vi "PicoScopeospaExampleRapidBlockBulkOverlapped_jittertimes.vi"() -> ()   [LabVIEW 2010]
uses:
  shared/PicoBuffers.ctl
  <vilib>/Waveform/DWDTOps.llb/DWDT Analog to Digital.vi
  PicoScopepsospaLib/PicoScopeospaDigitalChannelSettings.ctl
  PicoScopepsospaLib/PicoScopeospaAnalogChannelSettings.ctl
  shared/Buffer and Transfer Settings.ctl
  shared/Acquisition Settings.ctl
  shared/Segment Range.ctl
panel:
  out "nCaptures live":u64
  out "nCaptures":u64
  out "Trigger Info":T1(array[cluster])
  in  "timeIntervalRequested":dbl=2e-10 format="%#6_6p"
  in  "Write to file":bool
  in  "Channels":T2={"Channel A Settings "={"Enabled"=TRUE, "Coupling"=1, "Range"=8, "Analogue Offset"=0.0, "BandWidth"=0, "PROBE_RANGE_INFO"=0}, "Channel B Settings "={"Enabled"=FALSE, "Coupling"=1, "Range"=8, "Analogue Offset"=0.0, "BandWidth"=0, "PROBE_RANGE_INFO"=0}, "Channel C Settings "={"Enabled"=FALSE, "Coupling"=1, "Range"=8, "Analogue Offset"=0.0, "BandWidth"=0, "PROBE_RANGE_INFO"=0}, "Channel D Settings "={"Enabled"=FALSE, "Coupling"=1, "Range"=8, "Analogue Offset"=0.0, "BandWidth"=0, "PROBE_RANGE_INFO"=0}, "Channel E Settings "={"Enabled"=FALSE, "Coupling"=50, "Range"=5, "Analogue Offset"=0.0, "BandWidth"=0, "PROBE_RANGE_INFO"=0}, "Channel F Settings "={"Enabled"=FALSE, "Coupling"=50, "Range"=5, "Analogue Offset"=0.0, "BandWidth"=0, "PROBE_RANGE_INFO"=0}, "Channel G Settings "={"Enabled"=FALSE, "Coupling"=50, "Range"=5, "Analogue Offset"=0.0, "BandWidth"=0, "PROBE_RANGE_INFO"=0}, "Channel H Settings "={"Enabled"=FALSE, "Coupling"=50, "Range"=5, "Analogue Offset"=0.0, "BandWidth"=0, "PROBE_RANGE_INFO"=0}} {"Channel H Settings"."PROBE_RANGE_INFO" items=["PROBE_NONE_NV"=0, "X1_PROBE_NV"=1, "X10_PROBE_NV"=10]; "Channel H Settings"."BandWidth" items=["Full"=0, "100kHz"=100000, "20kHz"=200000, "1MHz"=1000000, "20MHz"=20000000, "25MHz"=25000000, "50MHz"=50000000, "200MHz"=200000000, "250MHz"=250000000, "500MHz"=500000000]; "Channel H Settings"."Range" items=["10mV"=0, "20mV"=1, "50mV"=2, "100mV"=3, "200mV"=4, "500mV"=5, "1V"=6, "2V"=7, "5V"=8, "10V"=9, "20V"=10, "50V"=11, "100V"=12, "200V"=13, "x10_Probe_100mV"=32, "x10_Probe_200mV"=33, "x10_Probe_500mV"=34, "x10_Probe_1V"=35, "x10_Probe_2V"=36, "x10_Probe_5V"=37, "x10_Probe_10V"=38, "x10_Probe_20V"=39, "x10_Probe_50V"=40, "x10_Probe_100V"=41, "x10_Probe_200V"=42, "x10_Probe_500V"=43, "CURRENT_CLAMP_60A_2A"=10500, "CURRENT_CLAMP_60A_5A"=10501, "CURRENT_CLAMP_60A_10A"=10502, "CURRENT_CLAMP_60A_20A"=10503, "CURRENT_CLAMP_60A_50A"=10504, "CURRENT_CLAMP_60A_60A"=10505, "CURRENT_CLAMP_60A_V2_0_5A"=10600, "CURRENT_CLAMP_60A_V2_1A"=10601, "CURRENT_CLAMP_60A_V2_2A"=10602, "CURRENT_CLAMP_60A_V2_5A"=10603, "CURRENT_CLAMP_60A_V2_10A"=10604, "CURRENT_CLAMP_60A_V2_20A"=10605, "CURRENT_CLAMP_60A_V2_50A"=10606, "CURRENT_CLAMP_60A_V2_60A"=10607, "RESISTANCE_LEAD_NEG5_TO_20OHM"=7000, "RESISTANCE_LEAD_NEG50_TO_200OHM"=7001, "RESISTANCE_LEAD_NEG500_TO_2KOHM"=7002, "RESISTANCE_LEAD_NEG5K_TO_20KOHM"=7003, "RESISTANCE_LEAD_NEG50K_TO_LEAD_200KOHM"=7004, "RESISTANCE_LEAD_NEG500K_TO_LEAD_2MOHM"=7005, "RESISTANCE_LEAD_DIODE_TEST"=7006, "HT_NEG3_TO_5KV"=8950, "HT_NEG3_TO_10KV"=8951, "HT_NEG5_TO_20KV"=8952, "HT_NEG5_TO_50KV"=8953, "HT_NEG5_TO_100KV"=8954, "HT_NEG3_TO_5KV_INVERTED"=8955, "HT_NEG3_TO_10KV_INVERTED"=8956, "HT_NEG5_TO_20KV_INVERTED"=8957, "HT_NEG5_TO_50KV_INVERTED"=8958, "HT_NEG5_TO_100KV_INVERTED"=8959, "TEMPERATURE_NEG50_TO_150DEGC"=9000, "PRESSURE_SENSOR_-100k-150k_PASCALS"=9100, "PRESSURE_SENSOR_-100k_TO_400k_PASCALS"=9101, "PRESSURE_SENSOR_-200k_TO_800k_PASCALS"=9102, "PRESSURE_SENSOR_-400k_TO_1600k_PASCALS"=9103, "PRESSURE_SENSOR_-400k_TO_3400k_PASCALS"=9104, "PRESSURE_SENSOR_-150k_TO_1350k_PASCALS"=9105]; "Channel H Settings"."Coupling" items=["AC"=0, "DC 1M Ohm"=1, "DC 50 Ohm"=50]; "Channel G Settings"."PROBE_RANGE_INFO" items=["PROBE_NONE_NV"=0, "X1_PROBE_NV"=1, "X10_PROBE_NV"=10]; "Channel G Settings"."BandWidth" items=["Full"=0, "100kHz"=100000, "20kHz"=200000, "1MHz"=1000000, "20MHz"=20000000, "25MHz"=25000000, "50MHz"=50000000, "200MHz"=200000000, "250MHz"=250000000, "500MHz"=500000000]; "Channel G Settings"."Range" items=["10mV"=0, "20mV"=1, "50mV"=2, "100mV"=3, "200mV"=4, "500mV"=5, "1V"=6, "2V"=7, "5V"=8, "10V"=9, "20V"=10, "50V"=11, "100V"=12, "200V"=13, "x10_Probe_100mV"=32, "x10_Probe_200mV"=33, "x10_Probe_500mV"=34, "x10_Probe_1V"=35, "x10_Probe_2V"=36, "x10_Probe_5V"=37, "x10_Probe_10V"=38, "x10_Probe_20V"=39, "x10_Probe_50V"=40, "x10_Probe_100V"=41, "x10_Probe_200V"=42, "x10_Probe_500V"=43, "CURRENT_CLAMP_60A_2A"=10500, "CURRENT_CLAMP_60A_5A"=10501, "CURRENT_CLAMP_60A_10A"=10502, "CURRENT_CLAMP_60A_20A"=10503, "CURRENT_CLAMP_60A_50A"=10504, "CURRENT_CLAMP_60A_60A"=10505, "CURRENT_CLAMP_60A_V2_0_5A"=10600, "CURRENT_CLAMP_60A_V2_1A"=10601, "CURRENT_CLAMP_60A_V2_2A"=10602, "CURRENT_CLAMP_60A_V2_5A"=10603, "CURRENT_CLAMP_60A_V2_10A"=10604, "CURRENT_CLAMP_60A_V2_20A"=10605, "CURRENT_CLAMP_60A_V2_50A"=10606, "CURRENT_CLAMP_60A_V2_60A"=10607, "RESISTANCE_LEAD_NEG5_TO_20OHM"=7000, "RESISTANCE_LEAD_NEG50_TO_200OHM"=7001, "RESISTANCE_LEAD_NEG500_TO_2KOHM"=7002, "RESISTANCE_LEAD_NEG5K_TO_20KOHM"=7003, "RESISTANCE_LEAD_NEG50K_TO_LEAD_200KOHM"=7004, "RESISTANCE_LEAD_NEG500K_TO_LEAD_2MOHM"=7005, "RESISTANCE_LEAD_DIODE_TEST"=7006, "HT_NEG3_TO_5KV"=8950, "HT_NEG3_TO_10KV"=8951, "HT_NEG5_TO_20KV"=8952, "HT_NEG5_TO_50KV"=8953, "HT_NEG5_TO_100KV"=8954, "HT_NEG3_TO_5KV_INVERTED"=8955, "HT_NEG3_TO_10KV_INVERTED"=8956, "HT_NEG5_TO_20KV_INVERTED"=8957, "HT_NEG5_TO_50KV_INVERTED"=8958, "HT_NEG5_TO_100KV_INVERTED"=8959, "TEMPERATURE_NEG50_TO_150DEGC"=9000, "PRESSURE_SENSOR_-100k-150k_PASCALS"=9100, "PRESSURE_SENSOR_-100k_TO_400k_PASCALS"=9101, "PRESSURE_SENSOR_-200k_TO_800k_PASCALS"=9102, "PRESSURE_SENSOR_-400k_TO_1600k_PASCALS"=9103, "PRESSURE_SENSOR_-400k_TO_3400k_PASCALS"=9104, "PRESSURE_SENSOR_-150k_TO_1350k_PASCALS"=9105]; "Channel G Settings"."Coupling" items=["AC"=0, "DC 1M Ohm"=1, "DC 50 Ohm"=50]; "Channel F Settings"."PROBE_RANGE_INFO" items=["PROBE_NONE_NV"=0, "X1_PROBE_NV"=1, "X10_PROBE_NV"=10]; "Channel F Settings"."BandWidth" items=["Full"=0, "100kHz"=100000, "20kHz"=200000, "1MHz"=1000000, "20MHz"=20000000, "25MHz"=25000000, "50MHz"=50000000, "200MHz"=200000000, "250MHz"=250000000, "500MHz"=500000000]; "Channel F Settings"."Range" items=["10mV"=0, "20mV"=1, "50mV"=2, "100mV"=3, "200mV"=4, "500mV"=5, "1V"=6, "2V"=7, "5V"=8, "10V"=9, "20V"=10, "50V"=11, "100V"=12, "200V"=13, "x10_Probe_100mV"=32, "x10_Probe_200mV"=33, "x10_Probe_500mV"=34, "x10_Probe_1V"=35, "x10_Probe_2V"=36, "x10_Probe_5V"=37, "x10_Probe_10V"=38, "x10_Probe_20V"=39, "x10_Probe_50V"=40, "x10_Probe_100V"=41, "x10_Probe_200V"=42, "x10_Probe_500V"=43, "CURRENT_CLAMP_60A_2A"=10500, "CURRENT_CLAMP_60A_5A"=10501, "CURRENT_CLAMP_60A_10A"=10502, "CURRENT_CLAMP_60A_20A"=10503, "CURRENT_CLAMP_60A_50A"=10504, "CURRENT_CLAMP_60A_60A"=10505, "CURRENT_CLAMP_60A_V2_0_5A"=10600, "CURRENT_CLAMP_60A_V2_1A"=10601, "CURRENT_CLAMP_60A_V2_2A"=10602, "CURRENT_CLAMP_60A_V2_5A"=10603, "CURRENT_CLAMP_60A_V2_10A"=10604, "CURRENT_CLAMP_60A_V2_20A"=10605, "CURRENT_CLAMP_60A_V2_50A"=10606, "CURRENT_CLAMP_60A_V2_60A"=10607, "RESISTANCE_LEAD_NEG5_TO_20OHM"=7000, "RESISTANCE_LEAD_NEG50_TO_200OHM"=7001, "RESISTANCE_LEAD_NEG500_TO_2KOHM"=7002, "RESISTANCE_LEAD_NEG5K_TO_20KOHM"=7003, "RESISTANCE_LEAD_NEG50K_TO_LEAD_200KOHM"=7004, "RESISTANCE_LEAD_NEG500K_TO_LEAD_2MOHM"=7005, "RESISTANCE_LEAD_DIODE_TEST"=7006, "HT_NEG3_TO_5KV"=8950, "HT_NEG3_TO_10KV"=8951, "HT_NEG5_TO_20KV"=8952, "HT_NEG5_TO_50KV"=8953, "HT_NEG5_TO_100KV"=8954, "HT_NEG3_TO_5KV_INVERTED"=8955, "HT_NEG3_TO_10KV_INVERTED"=8956, "HT_NEG5_TO_20KV_INVERTED"=8957, "HT_NEG5_TO_50KV_INVERTED"=8958, "HT_NEG5_TO_100KV_INVERTED"=8959, "TEMPERATURE_NEG50_TO_150DEGC"=9000, "PRESSURE_SENSOR_-100k-150k_PASCALS"=9100, "PRESSURE_SENSOR_-100k_TO_400k_PASCALS"=9101, "PRESSURE_SENSOR_-200k_TO_800k_PASCALS"=9102, "PRESSURE_SENSOR_-400k_TO_1600k_PASCALS"=9103, "PRESSURE_SENSOR_-400k_TO_3400k_PASCALS"=9104, "PRESSURE_SENSOR_-150k_TO_1350k_PASCALS"=9105]; "Channel F Settings"."Coupling" items=["AC"=0, "DC 1M Ohm"=1, "DC 50 Ohm"=50]; "Channel E Settings"."PROBE_RANGE_INFO" items=["PROBE_NONE_NV"=0, "X1_PROBE_NV"=1, "X10_PROBE_NV"=10]; "Channel E Settings"."BandWidth" items=["Full"=0, "100kHz"=100000, "20kHz"=200000, "1MHz"=1000000, "20MHz"=20000000, "25MHz"=25000000, "50MHz"=50000000, "200MHz"=200000000, "250MHz"=250000000, "500MHz"=500000000]; "Channel E Settings"."Range" items=["10mV"=0, "20mV"=1, "50mV"=2, "100mV"=3, "200mV"=4, "500mV"=5, "1V"=6, "2V"=7, "5V"=8, "10V"=9, "20V"=10, "50V"=11, "100V"=12, "200V"=13, "x10_Probe_100mV"=32, "x10_Probe_200mV"=33, "x10_Probe_500mV"=34, "x10_Probe_1V"=35, "x10_Probe_2V"=36, "x10_Probe_5V"=37, "x10_Probe_10V"=38, "x10_Probe_20V"=39, "x10_Probe_50V"=40, "x10_Probe_100V"=41, "x10_Probe_200V"=42, "x10_Probe_500V"=43, "CURRENT_CLAMP_60A_2A"=10500, "CURRENT_CLAMP_60A_5A"=10501, "CURRENT_CLAMP_60A_10A"=10502, "CURRENT_CLAMP_60A_20A"=10503, "CURRENT_CLAMP_60A_50A"=10504, "CURRENT_CLAMP_60A_60A"=10505, "CURRENT_CLAMP_60A_V2_0_5A"=10600, "CURRENT_CLAMP_60A_V2_1A"=10601, "CURRENT_CLAMP_60A_V2_2A"=10602, "CURRENT_CLAMP_60A_V2_5A"=10603, "CURRENT_CLAMP_60A_V2_10A"=10604, "CURRENT_CLAMP_60A_V2_20A"=10605, "CURRENT_CLAMP_60A_V2_50A"=10606, "CURRENT_CLAMP_60A_V2_60A"=10607, "RESISTANCE_LEAD_NEG5_TO_20OHM"=7000, "RESISTANCE_LEAD_NEG50_TO_200OHM"=7001, "RESISTANCE_LEAD_NEG500_TO_2KOHM"=7002, "RESISTANCE_LEAD_NEG5K_TO_20KOHM"=7003, "RESISTANCE_LEAD_NEG50K_TO_LEAD_200KOHM"=7004, "RESISTANCE_LEAD_NEG500K_TO_LEAD_2MOHM"=7005, "RESISTANCE_LEAD_DIODE_TEST"=7006, "HT_NEG3_TO_5KV"=8950, "HT_NEG3_TO_10KV"=8951, "HT_NEG5_TO_20KV"=8952, "HT_NEG5_TO_50KV"=8953, "HT_NEG5_TO_100KV"=8954, "HT_NEG3_TO_5KV_INVERTED"=8955, "HT_NEG3_TO_10KV_INVERTED"=8956, "HT_NEG5_TO_20KV_INVERTED"=8957, "HT_NEG5_TO_50KV_INVERTED"=8958, "HT_NEG5_TO_100KV_INVERTED"=8959, "TEMPERATURE_NEG50_TO_150DEGC"=9000, "PRESSURE_SENSOR_-100k-150k_PASCALS"=9100, "PRESSURE_SENSOR_-100k_TO_400k_PASCALS"=9101, "PRESSURE_SENSOR_-200k_TO_800k_PASCALS"=9102, "PRESSURE_SENSOR_-400k_TO_1600k_PASCALS"=9103, "PRESSURE_SENSOR_-400k_TO_3400k_PASCALS"=9104, "PRESSURE_SENSOR_-150k_TO_1350k_PASCALS"=9105]; "Channel E Settings"."Coupling" items=["AC"=0, "DC 1M Ohm"=1, "DC 50 Ohm"=50]; "Channel D Settings"."BandWidth" items=["Full"=0, "100kHz"=100000, "20kHz"=200000, "1MHz"=1000000, "20MHz"=20000000, "25MHz"=25000000, "50MHz"=50000000, "100MHz"=100000000, "200MHz"=200000000, "250MHz"=250000000, "350MHz"=350000000, "500MHz"=500000000]; "Channel D Settings"."PROBE_RANGE_INFO" items=["PROBE_NONE_NV"=0, "X1_PROBE_NV"=1, "X10_PROBE_NV"=10]; "Channel D Settings"."Range" items=["10mV", "20mV", "50mV", "100mV", "200mV", "500mV", "1V", "2V", "5V", "10V", "20V", "50V", "100V", "200V"]; "Channel D Settings"."Coupling" items=["AC"=0, "DC 1M Ohm"=1, "DC 50 Ohm"=50]; "Channel C Settings"."BandWidth" items=["Full"=0, "100kHz"=100000, "20kHz"=200000, "1MHz"=1000000, "20MHz"=20000000, "25MHz"=25000000, "50MHz"=50000000, "100MHz"=100000000, "200MHz"=200000000, "250MHz"=250000000, "350MHz"=350000000, "500MHz"=500000000]; "Channel C Settings"."PROBE_RANGE_INFO" items=["PROBE_NONE_NV"=0, "X1_PROBE_NV"=1, "X10_PROBE_NV"=10]; "Channel C Settings"."Range" items=["10mV", "20mV", "50mV", "100mV", "200mV", "500mV", "1V", "2V", "5V", "10V", "20V", "50V", "100V", "200V"]; "Channel C Settings"."Coupling" items=["AC"=0, "DC 1M Ohm"=1, "DC 50 Ohm"=50]; "Channel B Settings"."BandWidth" items=["Full"=0, "100kHz"=100000, "20kHz"=200000, "1MHz"=1000000, "20MHz"=20000000, "25MHz"=25000000, "50MHz"=50000000, "100MHz"=100000000, "200MHz"=200000000, "250MHz"=250000000, "350MHz"=350000000, "500MHz"=500000000]; "Channel B Settings"."PROBE_RANGE_INFO" items=["PROBE_NONE_NV"=0, "X1_PROBE_NV"=1, "X10_PROBE_NV"=10]; "Channel B Settings"."Range" items=["10mV", "20mV", "50mV", "100mV", "200mV", "500mV", "1V", "2V", "5V", "10V", "20V", "50V", "100V", "200V"]; "Channel B Settings"."Coupling" items=["AC"=0, "DC 1M Ohm"=1, "DC 50 Ohm"=50]; "Channel A Settings"."PROBE_RANGE_INFO" items=["PROBE_NONE_NV"=0, "X1_PROBE_NV"=1, "X10_PROBE_NV"=10]; "Channel A Settings"."Range" items=["10mV", "20mV", "50mV", "100mV", "200mV", "500mV", "1V", "2V", "5V", "10V", "20V", "50V", "100V", "200V"]; "Channel A Settings"."BandWidth" items=["Full"=0, "100kHz"=100000, "20kHz"=200000, "1MHz"=1000000, "20MHz"=20000000, "25MHz"=25000000, "50MHz"=50000000, "100MHz"=100000000, "200MHz"=200000000, "250MHz"=250000000, "350MHz"=350000000, "500MHz"=500000000]; "Channel A Settings"."Coupling" items=["AC"=0, "DC 1M Ohm"=1, "DC 50 Ohm"=50]}
  out "overflow":i16[](array[numeric])=[1023] format="%010d"
  out "Trigger Offsets":cluster{"Samples":u64, "Time (seconds)":dbl}[](array[cluster]) {"Time (seconds)" format="%#_5p"}
  in  "Stop Display":bool
  out "Capture Complete":bool
  in  "Run":bool
  in  "Display Buffer Index":i32
  in  "Segment Range":T3={"fromSegmentIndex"=0, "toSegmentIndex"=9} {"toSegmentIndex" format="%.4p"; "fromSegmentIndex" format="%.4p"}
  in  "nSegments":u64=10 format="%.4p"
  out "error out":errorcluster
  in  "Data file":path=path "PicoScopeospaExampleRapidBlock ChA Data"
  in  "Digital Channels":T4={"Port 0 Settings "={"Enabled"=FALSE, "Threshold Level (Volts)"=3.0}, "Port 1 Settings"={"Enabled"=FALSE, "Threshold Level (Volts)"=3.0}} {"Port 1 Settings"."Threshold Level (Volts)" format="%#_4p"; "Port 0 Settings"."Threshold Level (Volts)" format="%#_4p"}
  in  "Trigger Settings":T5={"Trigger Enabled"=FALSE, "Trigger Threshold (Volts)"=0.0, "Trigger Direction"=2, "Trigger Delay (samples)"=0, "Auto Trigger Time (us)"=1000000, "Trigger Source"=0} {"Trigger Source" items=["Channel A"=0, "Channel B"=1, "Channel C"=2, "Channel D"=3, "Channel E"=4, "Channel F"=5, "Channel G"=6, "Channel H"=7, "Port 0"=128, "Port 1"=129, "Trigger AUX"=1001]; "Auto Trigger Time (us)" format="%.4p"; "Trigger Direction" items=["Above", "Below", "Rising", "Falling", "Rising or Falling"]; "Trigger Threshold (Volts)" format="%#_6p"}
  in  "Buffer and Transfer Settings":T6={"startIndex"=0, "Samples"=10000000, "Down Sample Ratio"=10, "Down-Sample Mode"=2147483648} {"Down-Sample Mode" items=["RAW none"=2147483648, "None"=0, "Aggregate"=1, "Decimate"=2, "Average"=4]; "Down Sample Ratio" step=1; "Samples" format="%_6p"}
  in  "Acquisition Settings":T7={"preTriggerSamples"=0, "postTriggerSamples"=10000000, "timebase"=5} {"postTriggerSamples" format="%_6p"; "preTriggerSamples" format="%_6p"}
  out "Properties Panel":T8 {"Max Total Capture Time Available (sec)" format="%.3p"; "Sample Frequency" format="%.6p"; "Sample Rate" format="%.3p"; "Max Samples Available" format="%_6p"; "Total Capture Time (sec)" format="%.3p"}
  out "Port 0":digitalwaveform(graph)={"t0"=timestamp(0 s since 1904-01-01), "dt"=8e-09, "Y"={"transitions"=[], "data"=[]}}
  in  "stop":bool
  out "Analog Channels":cluster{i32, dbl, "Data":dbl[]}[](graph)
  out "Device Info":T9={"PICO_DRIVER_VERSION"="", "PICO_USB_VERSION"="", "PICO_HARDWARE_VERSION"="", "PICO_VARIANT_INFO"="", "PICO_BATCH_AND_SERIAL"="", "PICO_CAL_DATE"="", "PICO_KERNEL_VERSION"="", "PICO_DIGITAL_HARDWARE_VERSION"="", "PICO_ANALOGUE_HARDWARE_VERSION"="", "PICO_FIRMWARE_VERSION_1"="", "PICO_FIRMWARE_VERSION_2"="", "PICO_IPP_VERSION"="", "PICO_DRIVER_PATH"="", "PICO_FIRMWARE_VERSION_3"="", "PICO_FRONT_PANEL_FIRMWARE_VERSION"="", "Number of Channels"=8, "MSO"=FALSE}
  out "Pico ospa Units":string
  in  "Resolution":u32(ring)=10 items=["8-bit"=0, "12-bit"=1, "14-bit"=2, "15-bit"=3, "16-bit"=4, "10-bit"=10]
  in  "Serial Number":string
  in  "Use Serial Number":bool
  in  "error in (no error)":errorcluster
  # "Bit 0 = ChA"
  # "D8-D15"
  # "DO-D7"
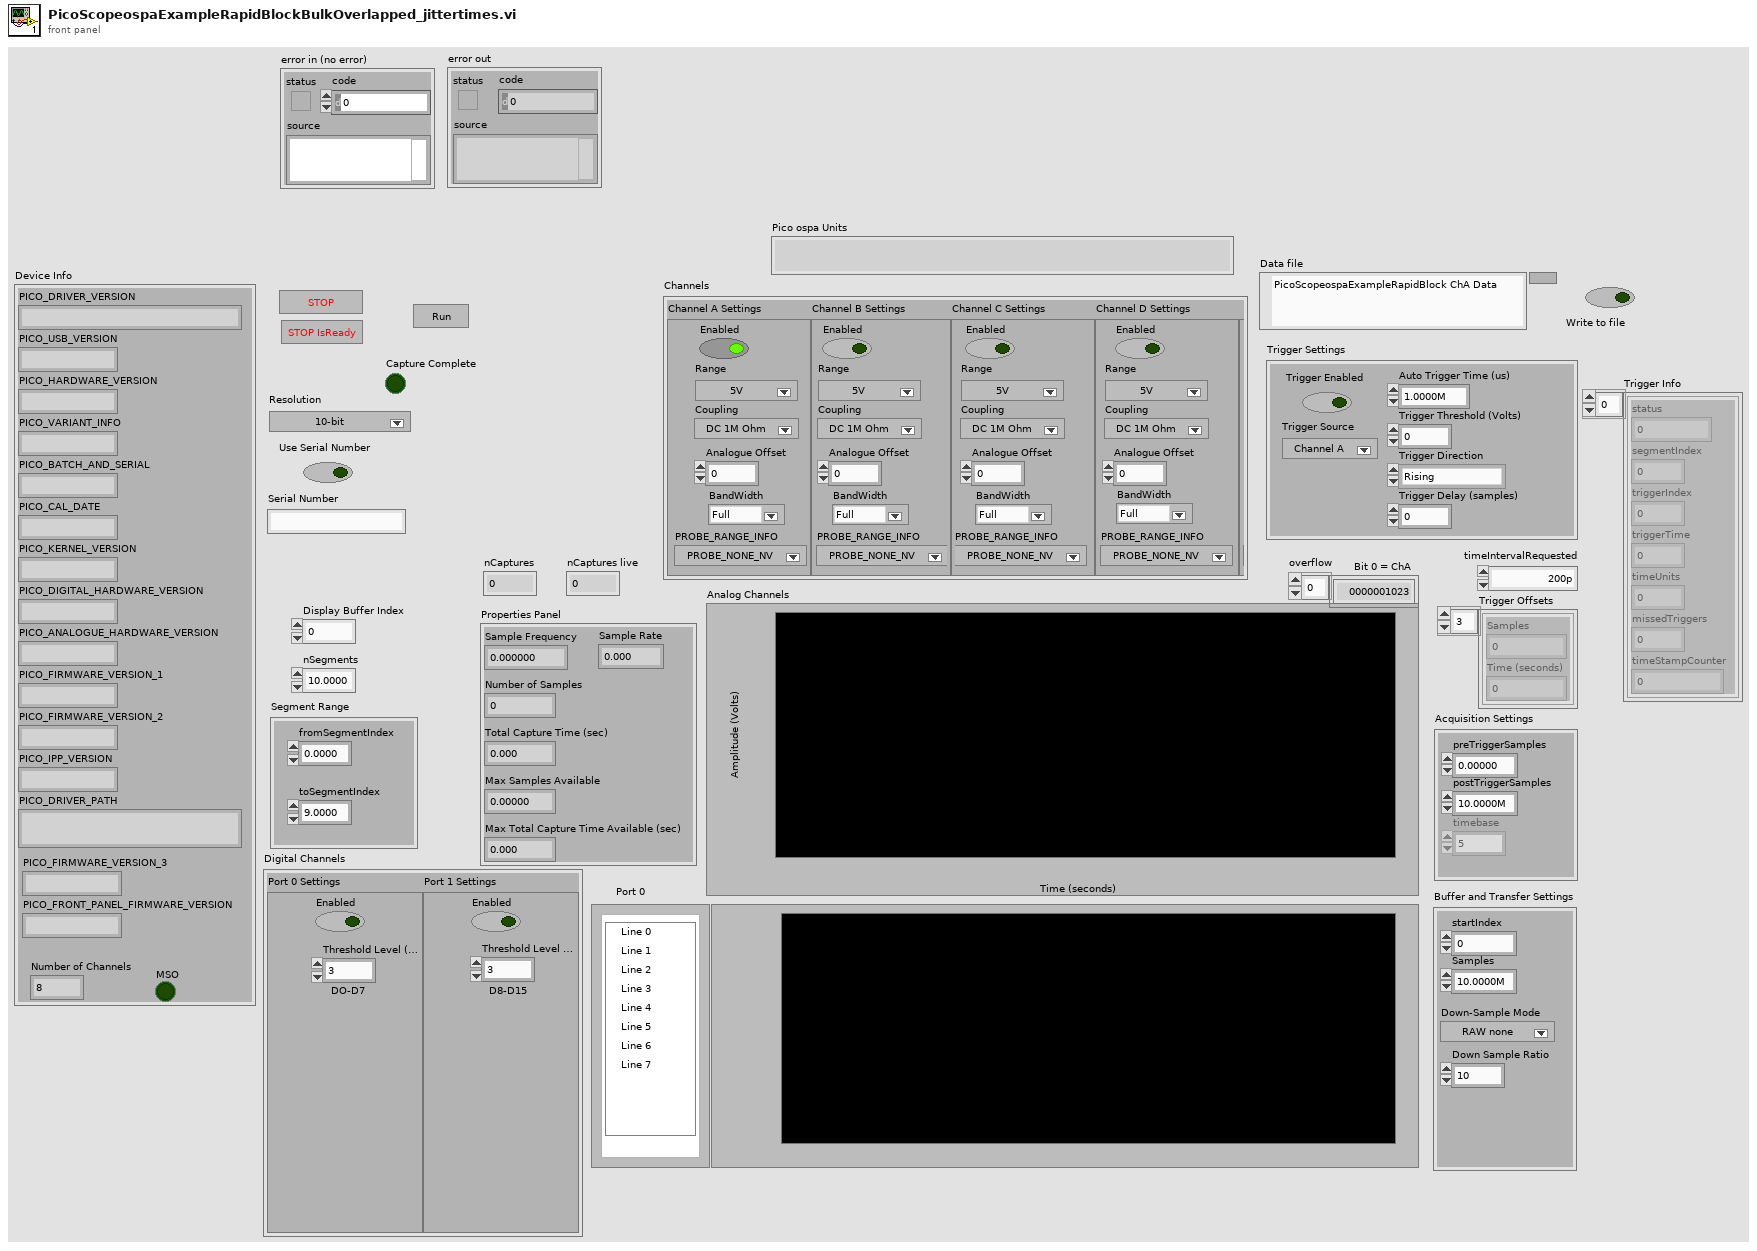
[diagram p1: front panel]
types:
  T1 = cluster{"status":u32, "segmentIndex":u64, "triggerIndex":u64, "triggerTime":dbl, "timeUnits":u32, "missedTriggers":u64, "timeStampCounter":u64}[]
  T2 = typedef "PicoScopeospaAnalogChannelSettings.ctl" = cluster{"Channel A Settings ":cluster{"Enabled":bool, "Coupling":i16, "Range":u16, "Analogue Offset":dbl, "BandWidth":u32, "PROBE_RANGE_INFO":u32}, "Channel B Settings ":cluster{"Enabled":bool, "Coupling":i16, "Range":u16, "Analogue Offset":dbl, "BandWidth":u32, "PROBE_RANGE_INFO":u32}, "Channel C Settings ":cluster{"Enabled":bool, "Coupling":i16, "Range":u16, "Analogue Offset":dbl, "BandWidth":u32, "PROBE_RANGE_INFO":u32}, "Channel D Settings ":cluster{"Enabled":bool, "Coupling":i16, "Range":u16, "Analogue Offset":dbl, "BandWidth":u32, "PROBE_RANGE_INFO":u32}, "Channel E Settings ":cluster{"Enabled":bool, "Coupling":i16, "Range":u16, "Analogue Offset":dbl, "BandWidth":u32, "PROBE_RANGE_INFO":u32}, "Channel F Settings ":cluster{"Enabled":bool, "Coupling":i16, "Range":u16, "Analogue Offset":dbl, "BandWidth":u32, "PROBE_RANGE_INFO":u32}, "Channel G Settings ":cluster{"Enabled":bool, "Coupling":i16, "Range":u16, "Analogue Offset":dbl, "BandWidth":u32, "PROBE_RANGE_INFO":u32}, "Channel H Settings ":cluster{"Enabled":bool, "Coupling":i16, "Range":u16, "Analogue Offset":dbl, "BandWidth":u32, "PROBE_RANGE_INFO":u32}}
  T3 = typedef "Segment Range.ctl" = cluster{"fromSegmentIndex":u64, "toSegmentIndex":u64}
  T4 = typedef "PicoScopeospaDigitalChannelSettings.ctl" = cluster{"Port 0 Settings ":cluster{"Enabled":bool, "Threshold Level (Volts)":dbl}, "Port 1 Settings":cluster{"Enabled":bool, "Threshold Level (Volts)":dbl}}
  T5 = cluster{"Trigger Enabled":bool, "Trigger Threshold (Volts)":dbl, "Trigger Direction":u16, "Trigger Delay (samples)":u64, "Auto Trigger Time (us)":u32, "Trigger Source":u32}
  T6 = typedef "Buffer and Transfer Settings.ctl" = cluster{"startIndex":u64, "Samples":u64, "Down Sample Ratio":u64, "Down-Sample Mode":u32}
  T7 = typedef "Acquisition Settings.ctl" = cluster{"preTriggerSamples":u64, "postTriggerSamples":u64, "timebase":u32}
  T8 = cluster{"Sample Frequency":dbl, "Sample Rate":dbl, "Max Samples Available":u64, "Number of Samples":u64, "Total Capture Time (sec) ":dbl, "Max Total Capture Time Available (sec)":dbl}
  T9 = cluster{"PICO_DRIVER_VERSION":string, "PICO_USB_VERSION":string, "PICO_HARDWARE_VERSION":string, "PICO_VARIANT_INFO":string, "PICO_BATCH_AND_SERIAL":string, "PICO_CAL_DATE":string, "PICO_KERNEL_VERSION":string, "PICO_DIGITAL_HARDWARE_VERSION":string, "PICO_ANALOGUE_HARDWARE_VERSION":string, "PICO_FIRMWARE_VERSION_1":string, "PICO_FIRMWARE_VERSION_2":string, "PICO_IPP_VERSION":string, "PICO_DRIVER_PATH":string, "PICO_FIRMWARE_VERSION_3":string, "PICO_FRONT_PANEL_FIRMWARE_VERSION":string, "Number of Channels":i16, "MSO":bool}
  T10 = typedef "PicoBuffers.ctl" = cluster{"Max Buffer Pointers":u64[][][], "Min Buffer Pointers":u64[][][], "StreamingDataInfo":cluster{"Channel":u32, "Down-Sample Mode":u32, "PICO_DATA_TYPE":enum32{"PICO_INT8_T", "PICO_INT16_T", "PICO_INT32_T", "PICO_UINT32_T", "PICO_INT64_T", ""}, "Samples":i32, "bufferIndex":u64, "startIndex":i32, "overflow":i16}[][]}
  T11 = enum16{"open", "open or create", "create or replace", "create", "open (read-only)"}
  T12 = cluster{"Channel A Buffer":i16[], "Channel B Buffer":i16[], "Channel C Buffer":i16[], "Channel D Buffer":i16[], "Channel E Buffer":i16[], "Channel F Buffer":i16[], "Channel G Buffer":i16[], "Channel H Buffer":i16[], "Port 0 Buffer":i16[], "Port 1 Buffer":i16[]}[]
  T13 = cluster{"Channel A Buffer":i16[], "Channel B Buffer":i16[], "Channel C Buffer":i16[], "Channel D Buffer":i16[], "Channel E Buffer":i16[], "Channel F Buffer":i16[], "Channel G Buffer":i16[], "Channel H Buffer":i16[], "Port 0 Buffer":i16[], "Port 1 Buffer":i16[]}
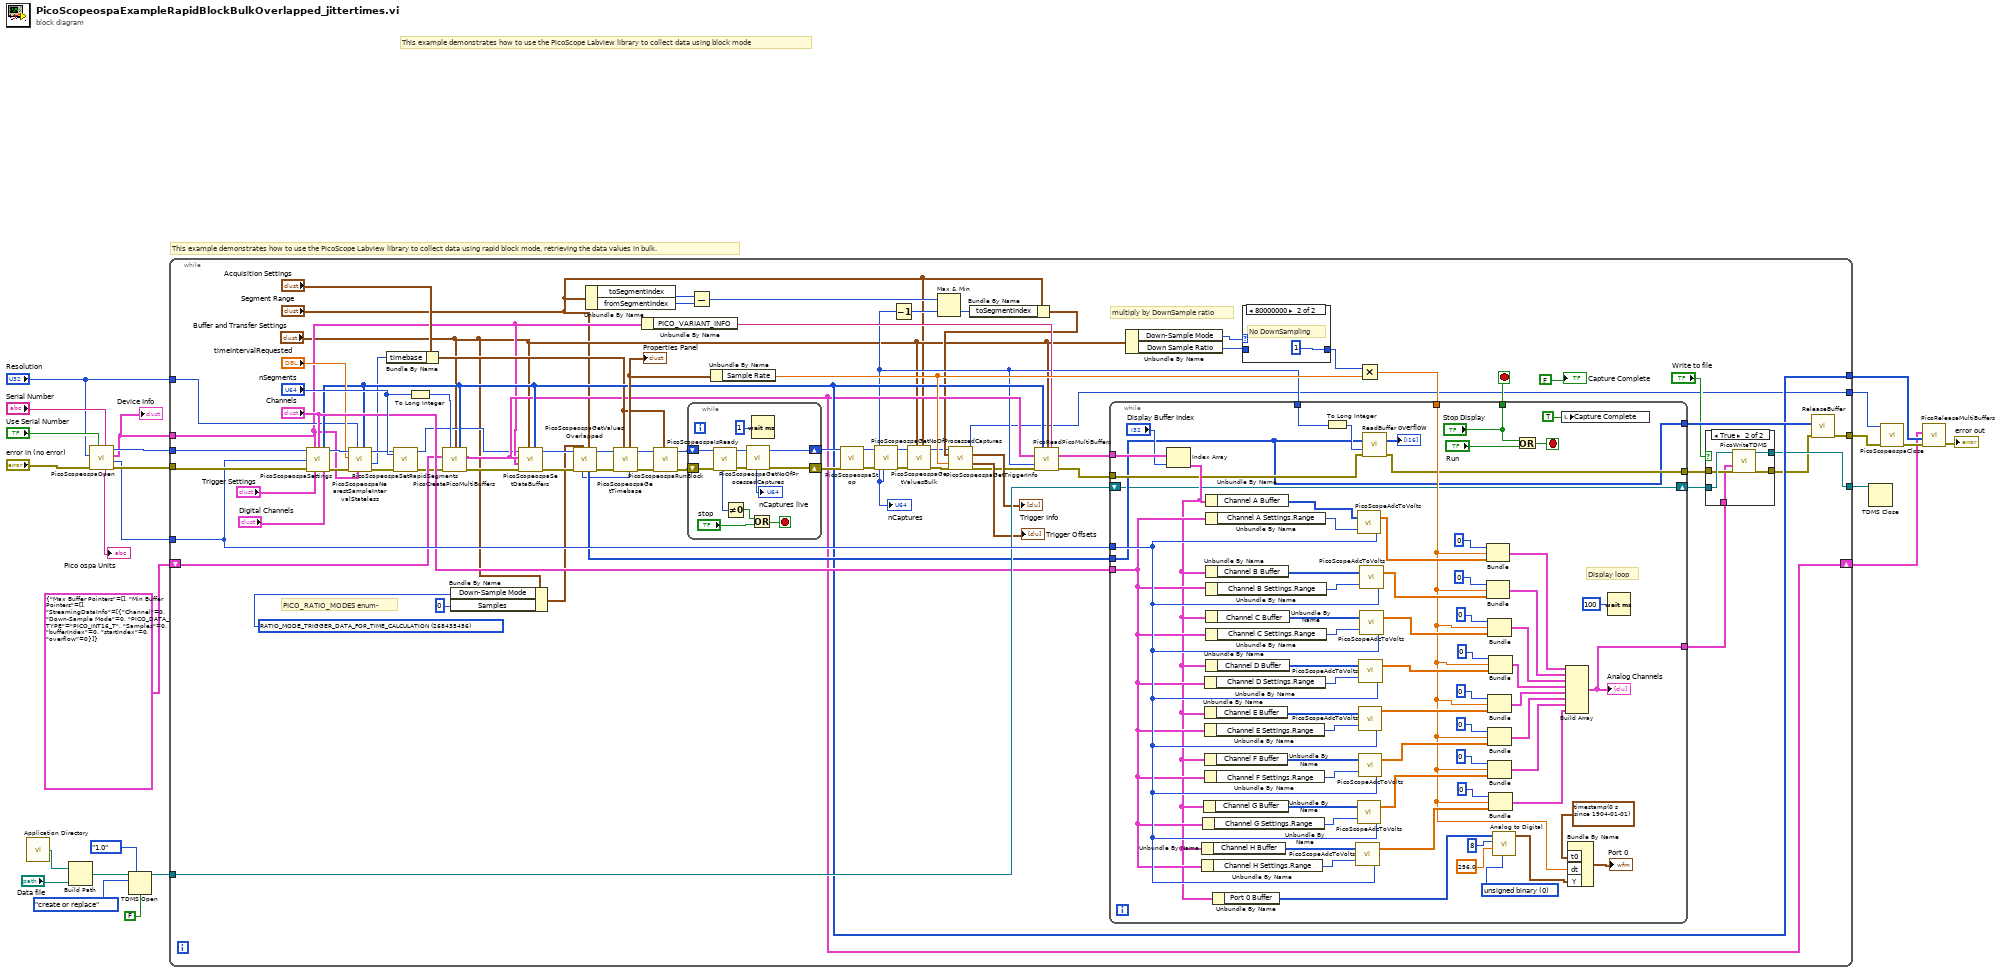
[diagram p0: block diagram]
diagram:
  # "This example demonstrates how to use the PicoScope Labview library to collect data using rapid block mode, retrieving the data values in bulk."
  # "This example demonstrates how to use the PicoScope Labview library to collect data using block mode"
  n1 = call <vilib>:"Application Directory.vi"() -> ("Application Directory"=w7:path)
  n2 = Build Path(base path=w7, name or relative path="Data file") -> (appended path=w8:path)
  n3 = call "PicoScopeospaOpen.vi"("Serial Number"="Serial Number", "Use Serial Number"="Use Serial Number", "error in (no error)"="error in (no error)", "Resolution"="Resolution") -> ("error out"=w20:errorcluster, "Max ADC value"=w18:i16, "Device Info"=w17:T9, "handle out"=w21:i16, "psospa Units"=→"Pico ospa Units":string)  [unwired: 2 in, 1 out]
  "Device Info" <- w17
  n4 = TDMS Open(6:FALSE ("disable buffering? (T)"), 7:enum16{"1.0", "2.0"}."1.0" ("file format version (2.0)"), 10:T11."create or replace" ("operation (0:open)"), 11:w8) -> (3:w5:refnum<k34>)  [unwired: 2 in, 1 out]
  n5 = while {
    tunnel: w17 -> [w47]
    tunnel: w18 -> [w100]
    tunnel: w21 -> [w102]
    tunnel: [w25] -> w14
    tunnel: w20 -> [w101]
    tunnel: [w67] -> w15
    tunnel: [w60] -> w16
    tunnel: [w51] -> w6
    tunnel: w5 -> [w96]
    tunnel: "Resolution" -> [w59]
    shift-right: [w48] -> w1
    shift-left: T10 {"Max Buffer Pointers"=[], "Min Buffer Pointers"=[], "StreamingDataInfo"=[[{"Channel"=0, "Down-Sample Mode"=0, "PICO_DATA_TYPE"=enum."PICO_INT16_T", "Samples"=0, "bufferIndex"=0, "startIndex"=0, "overflow"=0}]]} ("Data Pointers") -> [w49]
    stop <- w80 stop-if-true
    w36 = u32 268435456 items=["RAW none"=2147483648, "None"=0, "Aggregate"=1, "Decimate"=2, "Average"=4, "RATIO_MODE_TRIGGER_DATA_FOR_TIME_CALCULATION "=268435456, "PICO_RATIO_MODE_TRIGGER"=1073741824] ("Down-Sample Mode")
    # "PICO_RATIO_MODES enum-"
    # "multiply by DownSample ratio"
    n6 = call "PicoScopeospaSettings.vi"("handle in"=w102, "Device Info"=w47, "Channels"="Channels", "Max ADC value"=w100, "error in (no error)"=w101, "Trigger Settings"="Trigger Settings", "Digital Channels"="Digital Channels") -> ("Enabled array"=w60:i16[], "handle out"=w62:i16, "error out"=w65:errorcluster)  [unwired: 6 in]
    n7 = call "PicoScopeospaNearestSampleIntervalStateless.vi"("Enabled array"=w60, "Device Info"=w47, "Resolution"=w59, "error in (no error)"=w65, "timeIntervalRequested"="timeIntervalRequested", "handle in"=w62) -> ("error out"=w64:errorcluster, "timebase"=w58:u32, "handle out"=w63:i16)  [unwired: 2 in, 1 out]
    n8 = Bundle By Name(cluster="Acquisition Settings", "timebase"=w58) -> (w56:T7)
    n9 = call "PicoScopeospaSetRapidSegments.vi"("nSegments"="nSegments", "error in (no error)"=w64, "handle in"=w63) -> ("error out"=w46:errorcluster, "handle out"=w45:i16)  [unwired: 6 in, 1 out]
    n10 = To Long Integer(number="nSegments") -> (32bit integer=w92:i32)
    n11 = call "PicoCreatePicoMultiBuffers.vi"("Number of Buffers"=w92, "Buffer and Transfer Settings"="Buffer and Transfer Settings", "enabled array"=w60, "Data Pointers In"=w49, "error in (no error)"=w46) -> ("Data Pointers"=w48:T10, "error out"=w97:errorcluster)  [unwired: 9 in]
    n12 = Bundle By Name(cluster="Buffer and Transfer Settings", "Down-Sample Mode"=w36, "Samples"=u64 0) -> (w37:T6)
    n13 = call "PicoScopeospaSetDataBuffers.vi"("enabled array"=w60, "Buffer and Transfer Settings"="Buffer and Transfer Settings", "error in (no error)"=w97, "Device Info"=w47, "Data Pointers In"=w48, "handle in"=w45) -> ("error out"=w95:errorcluster, "handle out"=w94:i16)  [unwired: 4 in]
    n14 = call "PicoScopeospaGetValuesOverlapped.vi"("Segment Range"="Segment Range", "Buffer and Transfer Settings"=w37, "error in (no error)"=w95, "handle in"=w94) -> ("error out"=w78:errorcluster, "handle out"=w77:i16, "Pointer to Overflow"=w71:u64[], "noOfSamples"=w66:u64)  [unwired: 4 in]
    n15 = Unbundle By Name("Segment Range") -> ("toSegmentIndex"=w69:u64, "fromSegmentIndex"=w42:u64)
    n16 = call "PicoScopeospaGetTimebase.vi"("Number of Samples"=w66, "Acquisition Settings"=w56, "error in (no error)"=w78, "handle in"=w77) -> ("error out"=w84:errorcluster, "handle out"=w85:i16, "Properties Panel"=w88:T8)  [unwired: 5 in]
    "Properties Panel" <- w88
    n17 = Unbundle By Name(w47) -> ("PICO_VARIANT_INFO"=w72:string)
    n18 = call "PicoScopeospaRunBlock.vi"("Acquisition Settings"=w56, "error in (no error)"=w84, "handle in"=w85) -> ("error out"=w83:errorcluster, "handle out"=w82:i16)  [unwired: 5 in, 2 out]
    n19 = while {
      shift-right: [w178] -> w74
      shift-left: w83 -> [w187]
      shift-right: [w177] -> w73
      shift-left: w82 -> [w186]
      stop <- w184 stop-if-true
      n20 = call "PicoScopeospaIsReady.vi"("error in (no error)"=w187, "handle in"=w186) -> ("error out"=w180:errorcluster, "handle out"=w179:i16, "ready"=w185:i16)  [unwired: 7 in]
      n21 = Not Equal To 0?(x=w185) -> (x != 0?=w183:bool)
      n22 = call "PicoScopeospaGetNoOfProcessedCaptures.vi"("error in (no error)"=w180, "handle in"=w179) -> ("error out"=w178:errorcluster, "handle out"=w177:i16, "nCaptures"=→"nCaptures live":u64)  [unwired: 7 in]
      n23 = Or(x=w183, y="stop") -> (x .or. y?=w184:bool)
      n24 = Wait (ms)(milliseconds to wait=u32 1) -> ()  [unwired: 1 out]
    }
    n25 = Subtract(x=w69, y=w42) -> (x-y=w43:u64)
    n26 = Unbundle By Name(w88) -> ("Sample Rate"=w76:dbl)
    n27 = call "PicoScopeospaStop.vi"("error in (no error)"=w74, "handle in"=w73) -> ("error out"=w32:errorcluster, "handle out"=w31:i16)  [unwired: 8 in]
    n28 = call "PicoScopeospaGetNoOfProcessedCaptures.vi"("error in (no error)"=w32, "handle in"=w31) -> ("error out"=w30:errorcluster, "handle out"=w27:i16, "nCaptures"=w40:u64)  [unwired: 7 in]
    "nCaptures" <- w40
    n29 = Decrement(x=w40) -> (x-1=w41:u64)
    n30 = call "PicoScopeospaGetValuesBulk.vi"("Segment Range"="Segment Range", "Buffer and Transfer Settings"="Buffer and Transfer Settings", "error in (no error)"=w30, "handle in"=w27) -> ("error out"=w29:errorcluster, "handle out"=w28:i16)  [unwired: 4 in, 2 out]
    n31 = Max & Min(x=w43, y=w41) -> (min(x,y)=w39:u64)  [unwired: 1 out]
    n32 = Bundle By Name(cluster="Segment Range", "toSegmentIndex"=w39) -> (w38:T3)
    n33 = call "PicoScopeospaGetTriggerInfo.vi"("handle in"=w28, "Segment Range"=w38, "Sample Rate"=w76, "error in"=w29) -> ("handle out"=w25:i16, "Trigger Info"=→"Trigger Info":T1, "Trigger Offsets"=→"Trigger Offsets":cluster{"Samples":u64, "Time (seconds)":dbl}[], "error out"=w26:errorcluster)  [unwired: 8 in]
    n34 = call "PicoReadPicoMultiBuffers.vi"("enabled array"=w60, "Buffer and Transfer Settings"="Buffer and Transfer Settings", "Variant"=w72, "Data Pointers"=w48, "No of Buffers"=w40, "error in (no error)"=w26) -> ("MultiBuffers (Max or non-aggregated)"=w91:T12, "error out"=w81:errorcluster)  [unwired: 7 in, 1 out]
    n35 = Unbundle By Name("Buffer and Transfer Settings") -> ("Down-Sample Mode"=w89:u32, "Down Sample Ratio"=w90:u64)
    n36 = case shown="80000000" w89 {
      tunnel: [w188 u64 1 ("Down Sample Ratio")] -> w86
      tunnel: w90 -> [w188 _]
      frame Default {
      }
      frame -2147483648 {
        # "No DownSampling"
      }
    }
    n37 = Multiply(x=w86, y=w76) -> (x*y=w87:dbl)
    n38 = while {
      tunnel: w100 -> [w175]
      tunnel: "Channels" -> [w174]
      tunnel: w91 -> [w127]
      tunnel: w87 -> [w126]
      shift-right: [w111] -> w55
      shift-left: w96 -> [w111]
      tunnel: [w116] -> w54
      tunnel: w81 -> [w117]
      tunnel: ["Stop Display"] -> w80
      tunnel: w71 -> [w112]
      tunnel: w40 -> [w113]
      tunnel: [w112] -> w68
      tunnel: [w110] -> w52
      stop <- w120 stop-if-true
      w135 = u16 0 items=["unsigned binary", "offset binary", "2's complement"] ("data format (offset binary)")
      # "Display loop"
      n39 = Index Array(array=w127, index="Display Buffer Index") -> (element=w125:T13)
      n40 = Unbundle By Name(w125) -> ("Channel H Buffer"=w133:i16[])
      n41 = Unbundle By Name(w174) -> ("Channel H Settings.Range"=w155:u16)
      n42 = Unbundle By Name(w174) -> ("Channel G Settings.Range"=w156:u16)
      n43 = Unbundle By Name(w125) -> ("Channel G Buffer"=w157:i16[])
      n44 = Unbundle By Name(w174) -> ("Channel D Settings.Range"=w162:u16)
      n45 = Unbundle By Name(w125) -> ("Channel E Buffer"=w161:i16[])
      n46 = Unbundle By Name(w174) -> ("Channel E Settings.Range"=w160:u16)
      n47 = Unbundle By Name(w125) -> ("Channel F Buffer"=w159:i16[])
      n48 = Unbundle By Name(w174) -> ("Channel F Settings.Range"=w158:u16)
      n49 = Unbundle By Name(w125) -> ("Channel A Buffer"=w124:i16[])
      n50 = Unbundle By Name(w174) -> ("Channel A Settings.Range"=w172:u16)
      n51 = Unbundle By Name(w125) -> ("Channel B Buffer"=w170:i16[])
      n52 = Unbundle By Name(w125) -> ("Channel D Buffer"=w163:i16[])
      n53 = Unbundle By Name(w174) -> ("Channel B Settings.Range"=w169:u16)
      n54 = Unbundle By Name(w125) -> ("Channel C Buffer"=w165:i16[])
      n55 = Unbundle By Name(w174) -> ("Channel C Settings.Range"=w164:u16)
      n56 = Unbundle By Name(w125) -> ("Port 0 Buffer"=w132:i16[])
      n57 = To Long Integer(number=w113) -> (32bit integer=w114:i32)
      n58 = call "PicoScopeAdcToVolts.vi"("Max_adc"=w175, "Range Index"=w155, "Data"=w133) -> ("Data"=w150:dbl[])
      n59 = call "PicoScopeAdcToVolts.vi"("Max_adc"=w175, "Range Index"=w172, "Data"=w124) -> ("Data"=w128:dbl[])
      n60 = call "PicoScopeAdcToVolts.vi"("Max_adc"=w175, "Range Index"=w156, "Data"=w157) -> ("Data"=w144:dbl[])
      n61 = call "PicoScopeAdcToVolts.vi"("Max_adc"=w175, "Range Index"=w160, "Data"=w161) -> ("Data"=w147:dbl[])
      n62 = call "PicoScopeAdcToVolts.vi"("Max_adc"=w175, "Range Index"=w158, "Data"=w159) -> ("Data"=w143:dbl[])
      n63 = call "PicoScopeAdcToVolts.vi"("Max_adc"=w175, "Range Index"=w162, "Data"=w163) -> ("Data"=w148:dbl[])
      n64 = call "PicoScopeAdcToVolts.vi"("Max_adc"=w175, "Range Index"=w169, "Data"=w170) -> ("Data"=w168:dbl[])
      n65 = call "PicoScopeAdcToVolts.vi"("Max_adc"=w175, "Range Index"=w164, "Data"=w165) -> ("Data"=w149:dbl[])
      n66 = call "ReadBuffer.vi"("Pointer and BufferSize"=w112, "Buffer size"=w114, "error in (no error)"=w117) -> ("Output Array"=→"overflow":i16[], "error out"=w116:errorcluster)  [unwired: 11 in]
      n67 = Bundle(0, w126, "Data"=w128) -> (w167:cluster{i32, dbl, "Data":dbl[]})  [unwired: 1 in]
      n68 = Bundle(0, w126, "Data"=w168) -> (w166:cluster{i32, dbl, "Data":dbl[]})  [unwired: 1 in]
      n69 = Bundle(0, w126, "Data"=w149) -> (w142:cluster{i32, dbl, "Data":dbl[]})  [unwired: 1 in]
      n70 = Bundle(0, w126, "Data"=w147) -> (w140:cluster{i32, dbl, "Data":dbl[]})  [unwired: 1 in]
      n71 = Bundle(0, w126, "Data"=w143) -> (w139:cluster{i32, dbl, "Data":dbl[]})  [unwired: 1 in]
      n72 = Bundle(0, w126, "Data"=w144) -> (w138:cluster{i32, dbl, "Data":dbl[]})  [unwired: 1 in]
      n73 = Bundle(0, w126, "Data"=w148) -> (w141:cluster{i32, dbl, "Data":dbl[]})  [unwired: 1 in]
      n74 = Bundle(0, w126, "Data"=w150) -> (w137:cluster{i32, dbl, "Data":dbl[]})  [unwired: 1 in]
      n75 = call-poly <vilib>:"Analog to Digital.vi"("data format (offset binary)"=w135, "full-scale range (pk-pk)"=256.0, "resolution (16 bit)"=8, "analog waveform"=w132) -> ("digital waveform"=w129:digitalwaveform)  [unwired: 4 in, 3 out]
      n76 = Or(x="Stop Display", y="Run") -> (x .or. y?=w120:bool)
      n77 = local write "Capture Complete"(TRUE ("Capture Complete")) -> ()
      n78 = Build Array(w167, w166, w142, w141, w140, w139, w138, w137) -> (w110:cluster{i32, dbl, "Data":dbl[]}[])
      "Analog Channels" <- w110
      n79 = Bundle By Name("t0"=timestamp(0 s since 1904-01-01), "dt"=w126, "Y"=w129) -> (→"Port 0":digitalwaveform)  [unwired: 1 in]
      n80 = Wait (ms)(milliseconds to wait=u32 100) -> ()  [unwired: 1 out]
    }
    n81 = case shown="True" "Write to file" {
      tunnel: w55 -> [w103 w109]
      tunnel: w54 -> [w104 w108]
      tunnel: w52 -> [_ w107]
      tunnel: [w103 w106] -> w51
      tunnel: [w104 w105] -> w50
      frame False {
      }
      frame True {
        n82 = call "PicoWriteTDMS.vi"("error in (no error)"=w108, "Analog Channels"=w107, "Refnum in"=w109) -> ("error out"=w105:errorcluster, "Refnum out"=w106:refnum<k34>)  [unwired: 7 in]
      }
    }
    n83 = call "ReleaseBuffer.vi"("error in (no error)"=w50, "Pointer and BufferSize"=w68) -> ("error out"=w67:errorcluster)  [unwired: 9 in]
    "Capture Complete" <- FALSE ("Capture Complete")
  }
  n84 = TDMS Close(11:w6) -> ()  [unwired: 1 in, 2 out]
  n85 = call "PicoScopeospaClose.vi"("error in (no error)"=w15, "handle in"=w14) -> ("error out"=w13:errorcluster)  [unwired: 8 in, 1 out]
  n86 = call "PicoReleaseMultiBuffers.vi"("error in (no error)"=w13, "Enabled array"=w16, "Data Pointers"=w1) -> ("error out"=→"error out":errorcluster)  [unwired: 7 in, 1 out]
